vi "Func - Unload Functions.vi"(5 "unload all (F)":bool, 6 "error in":errorcluster, 8 "Array of func names":string[](array[string]), 9 "List of func names":string) -> (0 "error out":errorcluster)   [LabVIEW 2021]
doc: "This VI closes references to FuncVIs. Refer to the VI help for more details.\n\nPass function names to either the <b>Array of func names</b> control or the <b>List of func names</b> control. Note that this VI recognizes function names, not FuncVI names. To unload all FuncVIs, pass TRUE to the <b>unload all</b> control.\n\n::: CalcExpress Toolkit :::\nCopyright (c) 2000-2026 Konstantin Shifershteyn. All rights reserved."
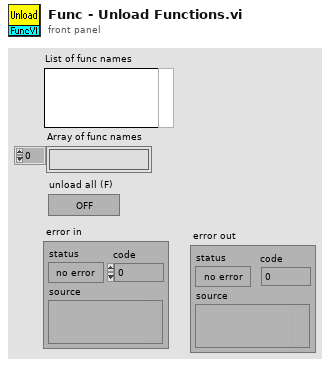
[diagram p1: front panel]
types:
  T1 = enum16{"get RefNum", "close Clones", "close RefNum", "close all RefNums", "update RefNums"}
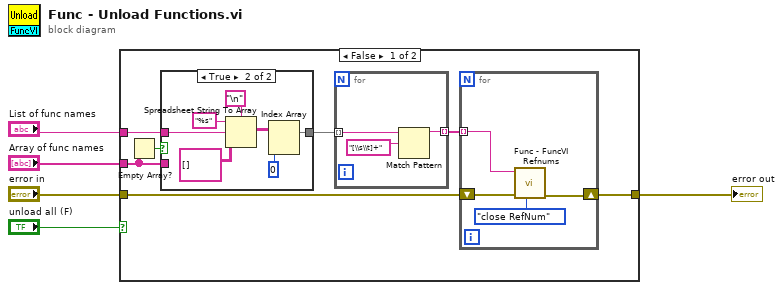
[diagram p0: block diagram]
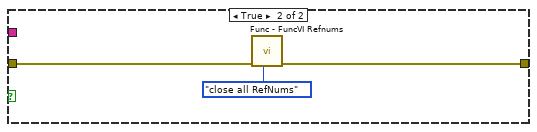
[diagram p3: hidden frame]
diagram:
  n1 = case shown="False" "unload all (F)" {
    tunnel: [w9 w29] -> w4
    tunnel: "error in" -> [w10 w30]
    tunnel: "List of func names" -> [w11 _]
    tunnel: "Array of func names" -> [w7 _]
    frame False {
      n2 = Empty Array?(array=w7) -> (empty?=w6:bool)
      n3 = case shown="True" w6 {
        tunnel: [w17 w20] -> w12
        tunnel: w7 -> [w17 _]
        tunnel: w11 -> [_ w22]
        frame False {
        }
        frame True {
          n4 = Spreadsheet String To Array(delimiter (Tab)="\n", format string="%s", spreadsheet string=w22, array type (2D Dbl)=string[][] []) -> (array=w21:string[][])
          n5 = Index Array(array=w21, index (col)=0) -> (element=w20:string[])  [unwired: 1 in]
        }
      }
      n6 = for {
        tunnel: [w26] -> w8 mode=indexing
        tunnel: w12 -> [w25] mode=indexing
        n7 = Match Pattern(string=w25, regular expression="[\\s\\t]+") -> (before substring=w26:string)  [unwired: 1 in, 3 out]
      }
      n8 = for {
        tunnel: w8 -> [w14] mode=indexing
        shift-right: [w15] -> w9
        shift-left: w10 -> [w16]
        n9 = call "Func - FuncVI Refnums.vi"("cmd (get)"=T1."close RefNum", "error in"=w16, "Func name"=w14) -> ("error out"=w15:errorcluster)  [unwired: 4 in, 4 out]
      }
    }
    frame True {
      n10 = call "Func - FuncVI Refnums.vi"("cmd (get)"=T1."close all RefNums", "error in"=w30) -> ("error out"=w29:errorcluster)  [unwired: 5 in, 4 out]
    }
  }
  "error out" <- w4
